vi "Launch Message Counter.vi"() -> ()   [LabVIEW 2026]
doc: "Beginner Actor Framework example. Run this VI. Send Add or Reset messages; Count is owned by CounterActor. Stop or window close sends the normal stop message and waits for Stop Core notification. No hardware required."
uses:
  CounterActor/CounterActor.lvclass
  C:/Program Files/National Instruments/LabVIEW 2026/vi.lib/ActorFramework/Actor/Actor.lvclass
  <vilib>/ActorFramework/Message Enqueuer/Message Enqueuer.lvclass/Message Enqueuer.ctl
  <vilib>/ActorFramework/Message Enqueuer/Enqueue.vi
  <vilib>/ActorFramework/Stop Msg/Stop Msg.lvclass
  C:/Program Files/National Instruments/LabVIEW 2026/vi.lib/ActorFramework/Message/Message.lvclass
  <vilib>/ActorFramework/Message Priority Queue/Priority Enqueue.vi
  <vilib>/ActorFramework/Actor/Actor.lvclass
  Messages/Add/Counter Add Msg.lvclass
  Messages/Reset/Counter Reset Msg.lvclass
panel:
  out "error out":errorcluster
  in  "Stop":bool
  in  "Reset":bool
  in  "Delta":dbl=1.0
  in  "Send Add":bool
  out "Stopped cleanly":bool
  out "Processed":dbl
  out "Count":dbl
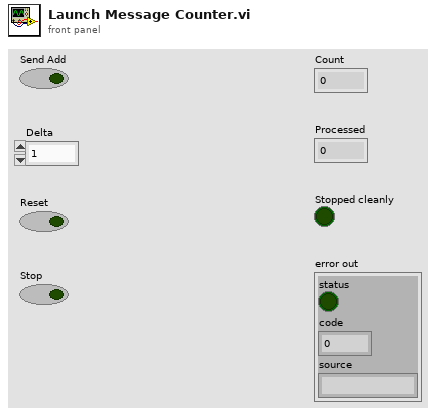
[diagram p1: front panel]
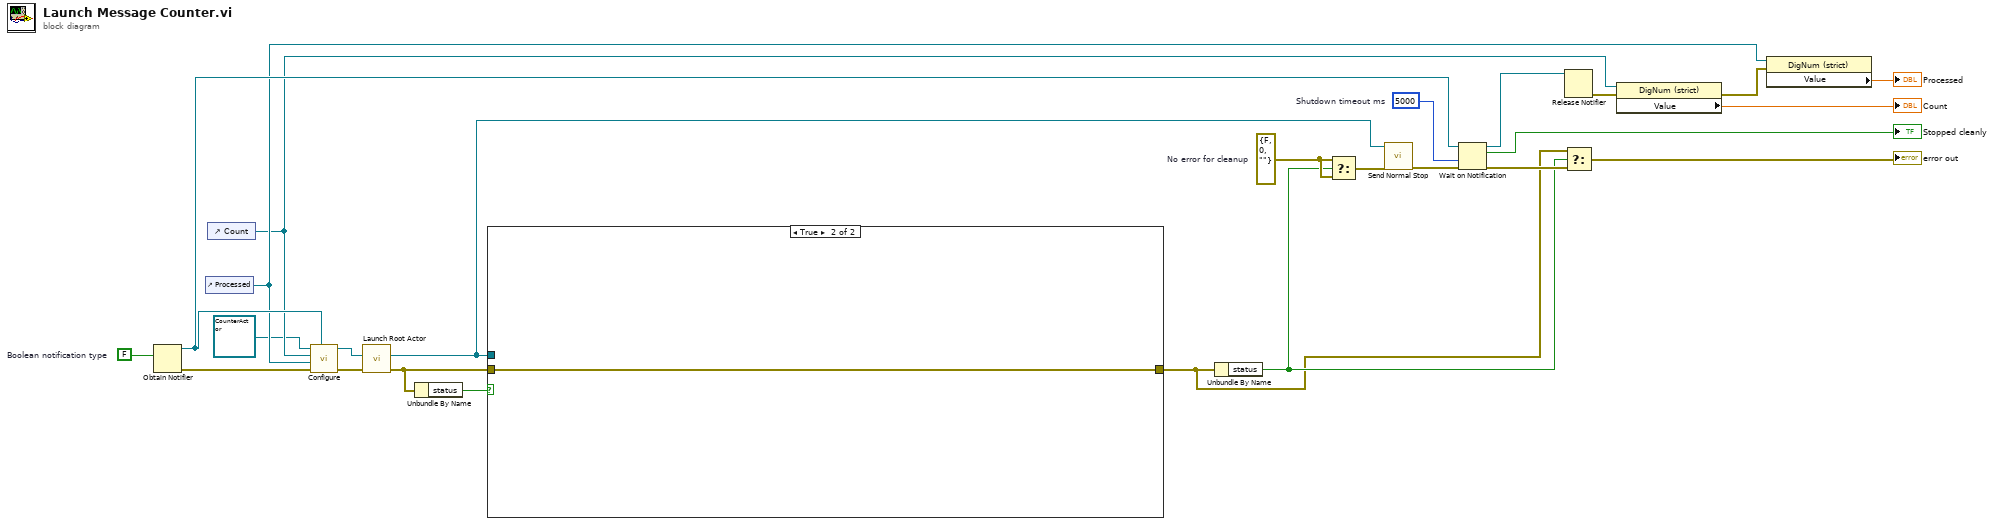
[diagram p0: block diagram]
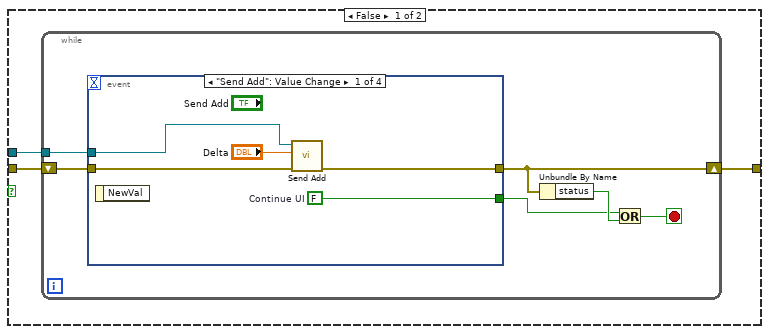
[diagram p2: hidden frame]
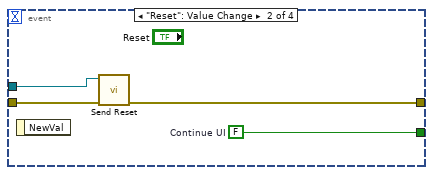
[diagram p3: hidden frame]
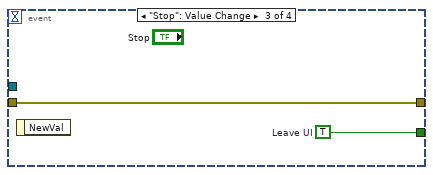
[diagram p4: hidden frame]
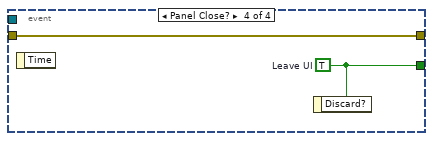
[diagram p5: hidden frame]
diagram:
  w20 = 5000  # Shutdown timeout ms
  w19 = errorcluster {"status"=FALSE, "code"=0, "source"=""}  # No error for cleanup
  w7 = FALSE  # Boolean notification type
  n1 = Obtain Notifier(notification data type=w7) -> (notifier out=w8:refnum<notifier>, error out=w9:errorcluster)  [unwired: 3 in, 1 out]
  n2 = control-ref of="Processed"() -> (w6:refnum<vi>)
  n3 = control-ref of="Count"() -> (w5:refnum<vi>)
  n4 = call "Configure.vi"("Stopped Notification"=w8, "error in"=w9, "Processed Display"=w6, "Count Display"=w5, "Actor in"=refnum<class "CounterActor.lvclass"> refnum ("CounterActor")) -> ("error out"=w11:errorcluster, "Actor out"=w10:refnum<class "CounterActor.lvclass">)  [unwired: 5 in]
  n5 = call <vilib>:"Launch Root Actor.vi"("error in (no error)"=w11, "Actor"=w10) -> ("error out"=w13:errorcluster, "Actor's Enqueuer"=w12:refnum<class "Message Enqueuer.lvclass">)  [unwired: 8 in]
  n6 = Unbundle By Name(w13) -> ("status"=w14:bool)
  n7 = case shown="True" w14 {
    tunnel: w12 -> [w26 _]
    tunnel: w13 -> [w27 w48]
    tunnel: [w28 w48] -> w15
    frame False {
      n8 = while {
        tunnel: w26 -> [w29]
        shift-right: [w31] -> w28
        shift-left: w27 -> [w30]
        stop <- w34 stop-if-true
        n9 = event shown="[0] \"Send Add\": Value Change" {
          selector: _ -> [_ _ _ _]
          dyn-events: _ -> [_ _ _ _]
          timeout: _ -> [_ _ _ _]
          tunnel: [w37 w42 w45 w47] -> w32
          tunnel: w29 -> [w35 w40 _ _]
          tunnel: w30 -> [w36 w41 w44 w46]
          tunnel: [w39 w43 w44 w46] -> w31
          event "Send Add": Value Change {
            w37 = FALSE  # Continue UI
            n10 = event-data() -> ()  [unwired: 1 in, 1 out]
            n11 = call "Send Add.vi"("error in (no error)"=w36, "Delta"="Delta", "Message Enqueuer"=w35) -> ("error out"=w39:errorcluster)  [unwired: 7 in, 1 out]
          }
          event "Reset": Value Change {
            w42 = FALSE  # Continue UI
            n12 = event-data() -> ()  [unwired: 1 in, 1 out]
            n13 = call "Send Reset.vi"("error in (no error)"=w41, "Message Enqueuer"=w40) -> ("error out"=w43:errorcluster)  [unwired: 8 in, 1 out]
          }
          event "Stop": Value Change {
            w45 = TRUE  # Leave UI
            n14 = event-data() -> ()  [unwired: 1 in, 1 out]
          }
          event Panel Close? {
            w47 = TRUE  # Leave UI
            n15 = event-data() -> ()  [unwired: 1 in, 1 out]
            n16 = event-data("Discard?"=w47) -> ()  [unwired: 1 in, 1 out]
          }
        }
        n17 = Unbundle By Name(w31) -> ("status"=w33:bool)
        n18 = Or(x=w32, y=w33) -> (x .or. y?=w34:bool)
      }
    }
    frame True {
    }
  }
  n19 = Unbundle By Name(w15) -> ("status"=w18:bool)
  n20 = Select(t=w19, s=w18, f=w19) -> (s? t:f=w17:errorcluster)
  n21 = call <vilib>:"Send Normal Stop.vi"("error in (no error)"=w17, "Message Enqueuer"=w12) -> ("error out"=w16:errorcluster)  [unwired: 9 in]
  n22 = Wait on Notification(notifier=w8, timeout in ms (-1)=w20, error in (no error)=w16) -> (notifier out=w21:refnum<notifier>, notification=→"Stopped cleanly":bool, error out=w22:errorcluster)  [unwired: 1 in, 1 out]
  n23 = Release Notifier(notifier=w21) -> (error out=w23:errorcluster)  [unwired: 2 in, 2 out]
  n24 = Select(t=w15, s=w18, f=w22) -> (s? t:f=→"error out":errorcluster)
  n25 = property class="DigNum (strict)"(reference=w5, error in=w23) -> (error out=w24:errorcluster, "Value"=→"Count":dbl)  [unwired: 1 out]
  n26 = property class="DigNum (strict)"(reference=w6, error in=w24) -> ("Value"=→"Processed":dbl)  [unwired: 2 out]
